vi "TEST - Wait (ms).vi"(8 "error in (no error)":errorcluster) -> (0 "error out":errorcluster, 2 "pass":bool)   [LabVIEW 2020]
uses:
  <vilib>/addons/_JKI Toolkits/Caraya/classes/Assert/Assert True.vi
  source/library/openg_time.lvlib
  <vilib>/addons/_JKI Toolkits/Caraya/classes/Test/Test.lvclass
  <vilib>/addons/_JKI Toolkits/Caraya/classes/Assert/Assert.lvclass
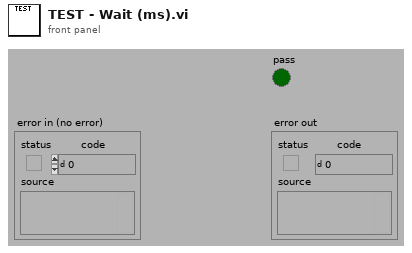
[diagram p1: front panel]
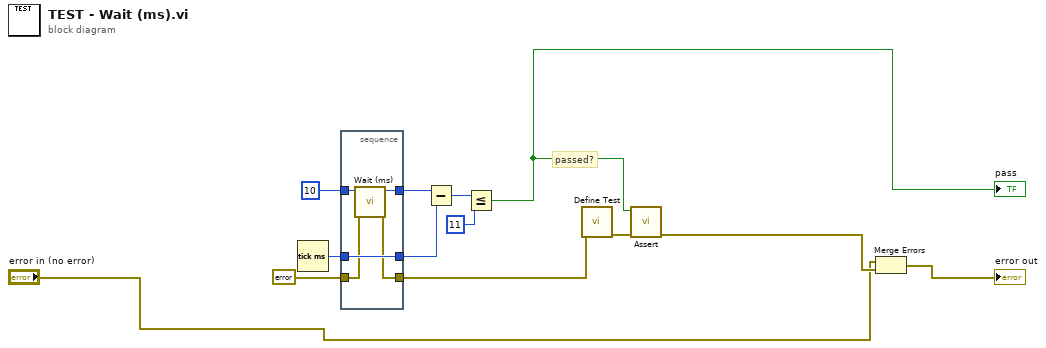
[diagram p0: block diagram]
diagram:
  # "passed?"
  n1 = Tick Count (ms)() -> (millisecond timer value=w9:u32)
  n2 = stacked-sequence {
    tunnel: [w16] -> w3
    tunnel: errorcluster {"status"=FALSE, "code"=0, "source"=""} ("error IO") -> [w17]
    tunnel: [w15] -> w11
    tunnel: [w18] -> w10
    tunnel: w9 -> [w18]
    tunnel: u32 10 ("milliseconds to wait") -> [w14]
    frame #0 {
      n3 = call "Wait (ms).vi"("error in (no error)"=w17, "milliseconds to wait"=w14) -> ("error out"=w16:errorcluster, "millisecond timer value"=w15:u32)  [unwired: 8 in]
    }
  }
  n4 = Subtract(x=w11, y=w10) -> (x-y=w8:u32)
  n5 = Less Or Equal?(x=w8, y=u32 11) -> (x <= y?=w13:bool)
  "pass" <- w13
  n6 = call <vilib>:"Define Test.vi"("error in (no error)"=w3) -> ("error out"=w5:errorcluster)  [unwired: 9 in, 1 out]
  n7 = call-poly <vilib>:"Assert.vi"("error in (no error)"=w5, "True?"=w13) -> ("error out"=w2:errorcluster)  [unwired: 8 in, 1 out]
  n8 = Merge Errors("error in (no error)", w2) -> (→"error out":errorcluster)
